vi "thermal_optical_capture_12.vi"() -> ()   [LabVIEW 2025]
panel:
  out "Optical saving error":errorcluster
  out "Thermal Preview":T1(plugin-control)
  in  "Stop Preview":bool
  out "Times between Frames":u32
  in  "STOP ACQUISITION":bool
  out "Optical Frame Out":string
  out "Optical Preview":T1(plugin-control)
  in  "Focus":dbl(slide) scale=0.0..100.0
  out "Thermal Frame Out":string
  in  "Output Folder":path
  in  "thermal capture interval (s)":dbl
  in  "Flag Button":bool
  in  "Stop & Save":bool
  in  "Record":bool
  # "Thermal Record"
  # "(Enter \"28\")"
  # "^ append to base data folder \"...\\test_n\\raw\" for nth recording"
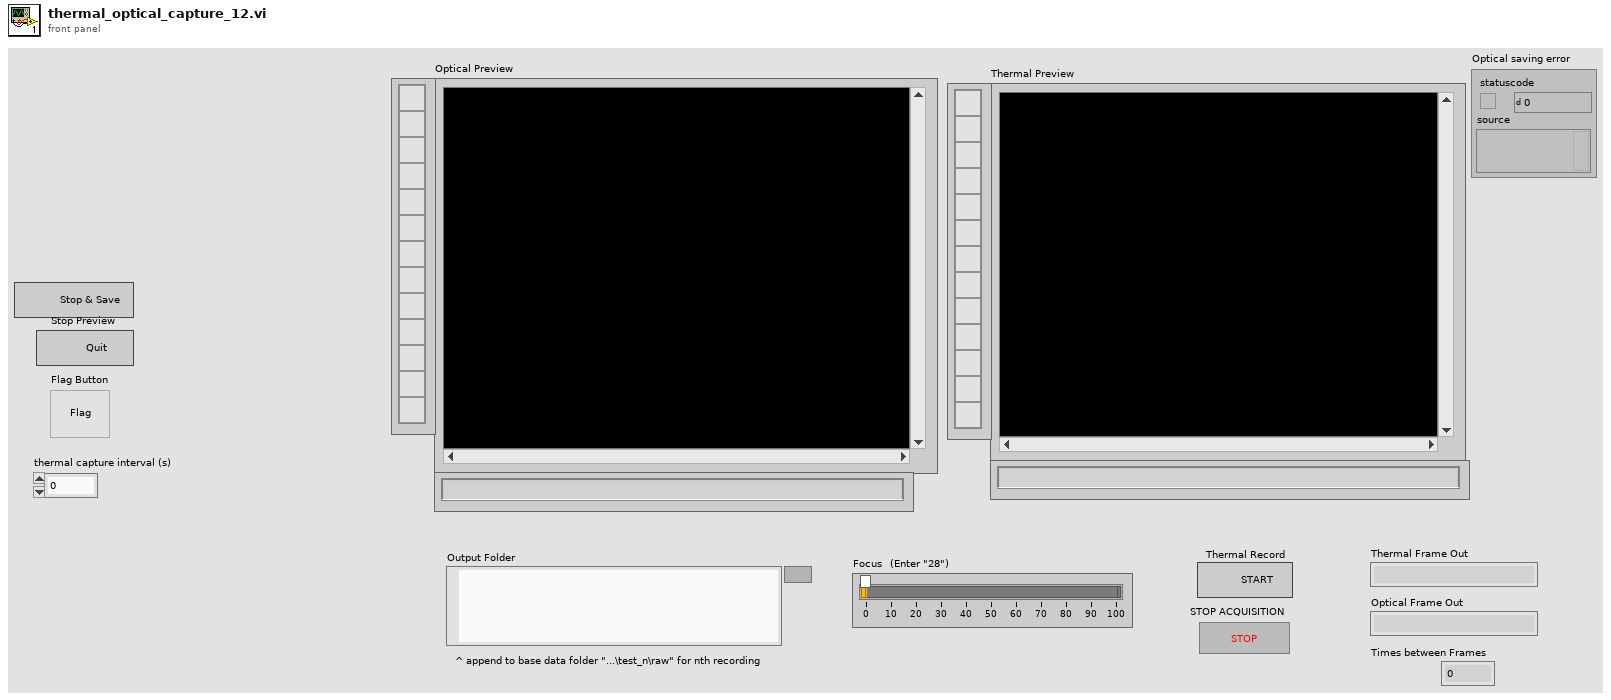
[diagram p1: front panel]
types:
  T1 = typedef "IMAQ Image.ctl" = refnum<image>
  T2 = enum16{"open", "replace", "create", "open or create", "replace or create", "replace or create with confirmation"}
  T3 = enum16{"big-endian, network order", "native, host order", "little-endian"}
  T4 = typedef "Image Type" = u32
  T5 = enum16{"Standard", "Buffered", "CRLF", "Immediate"}
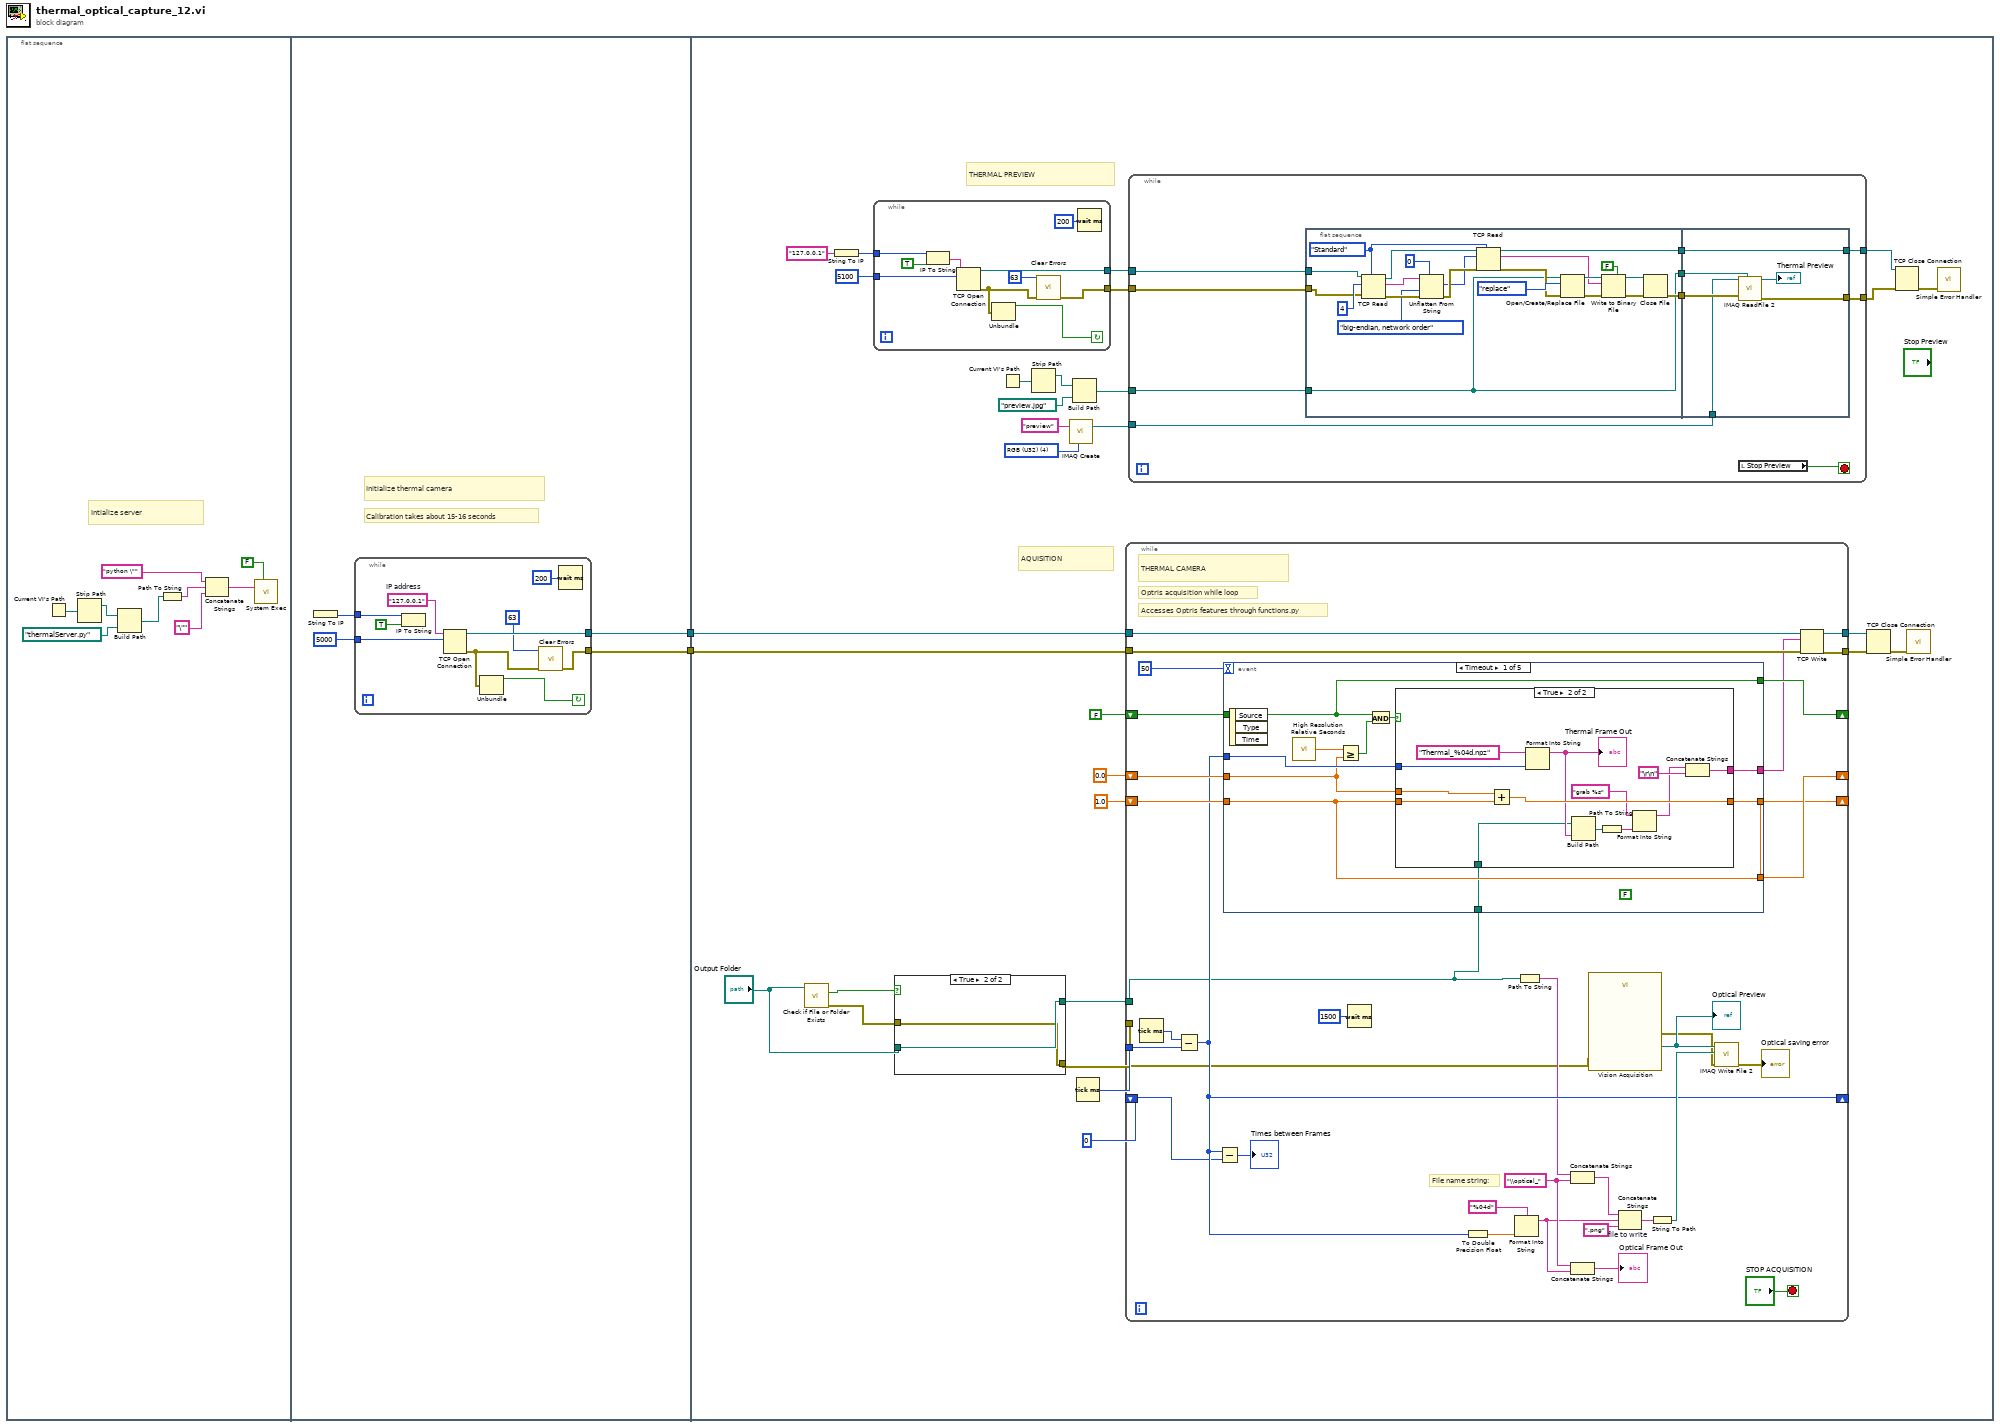
[diagram p0: block diagram]
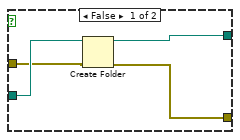
[diagram p2: hidden frame]
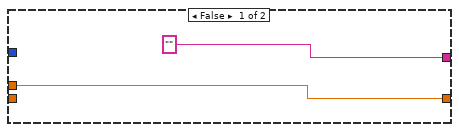
[diagram p3: hidden frame]
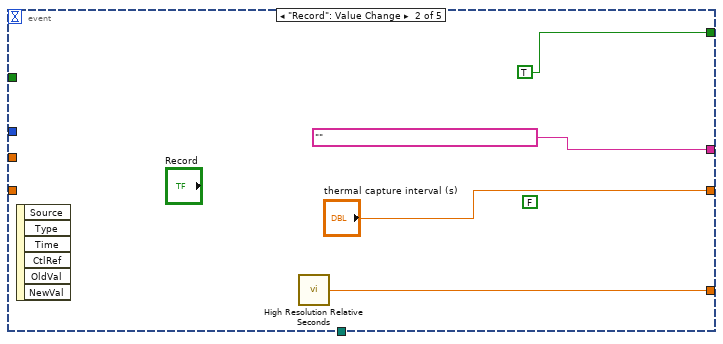
[diagram p4: hidden frame]
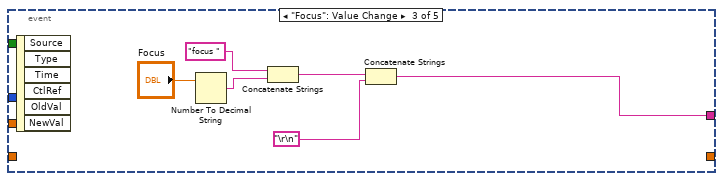
[diagram p5: hidden frame]
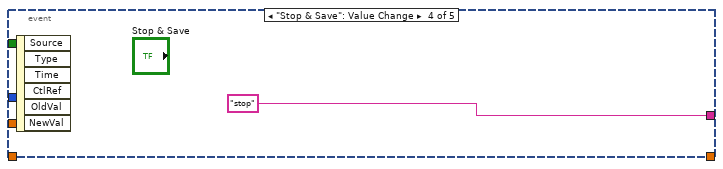
[diagram p6: hidden frame]
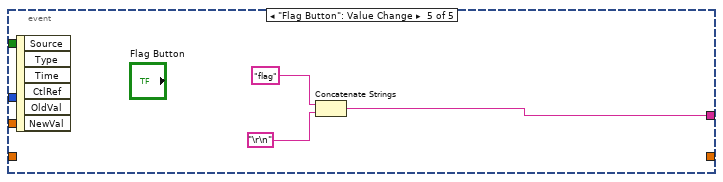
[diagram p7: hidden frame]
diagram:
  n1 = flat-sequence {
    tunnel: [w13] -> w2
    tunnel: [w12] -> w1
    tunnel: w1 -> [w52]
    tunnel: w2 -> [w51]
    frame #0 {
      # "Intialize server"
      n2 = Current VI's Path() -> (path=w6:path)
      n3 = Strip Path(path=w6) -> (stripped path=w7:path)  [unwired: 1 out]
      n4 = Build Path(base path=w7, name or relative path=path "thermalServer.py") -> (appended path=w4:path)
      n5 = Path To String(path=w4) -> (string=w10:string)
      n6 = Concatenate Strings("python \"" ("string"), w10, "\"" ("string")) -> (w9:string)
      n7 = call <vilib>:"System Exec.vi"("wait until completion? (T)"=FALSE, "command line"=w9) -> ()  [unwired: 6 in, 4 out]
    }
    frame #1 {
      # "Initialize thermal camera"
      # "Calibration takes about 15-16 seconds"
      n8 = String To IP() -> (0:w15:u32)  [unwired: 1 in]
      n9 = while {
        tunnel: [w20] -> w13
        tunnel: [w25] -> w12
        tunnel: w15 -> [w24]
        tunnel: u16 5000 ("remote port or service name") -> [w22]
        stop <- w17 continue-if-true
        w16 = "127.0.0.1"  # IP address
        n10 = IP To String(1:TRUE ("dot notation? (F)"), 2:w24) -> ()  [unwired: 1 out]
        n11 = TCP Open Connection(address=w16, remote port or service name=w22) -> (connection ID=w25:refnum<k5>, error out=w21:errorcluster)  [unwired: 3 in]
        n12 = Unbundle(w21) -> ("status"=w17:bool)  [unwired: 2 out]
        n13 = call <vilib>:"Clear Errors.vi"("error in (no error)"=w21, "specific error code to clear (0: all)"=63) -> ("error out"=w20:errorcluster)  [unwired: 4 in, 1 out]
        n14 = Wait (ms)(milliseconds to wait=u32 200) -> ()  [unwired: 1 out]
      }
    }
    frame #2 {
      w36 = T4 4 items=["Grayscale (U8)", "Grayscale (I16)", "Grayscale (SGL)", "Complex (CSG)", "RGB (U32)", "HSL (U32)", "RGB (U64)", "Grayscale (U16)"] ("Image Type")
      # "THERMAL PREVIEW"
      # "AQUISITION"
      n15 = call <vilib>:"Check if File or Folder Exists.vi"("path"="Output Folder") -> ("error out"=w27:errorcluster, "file or folder exists?"=w30:bool)  [unwired: 8 in, 1 out]
      n16 = String To IP(1:"127.0.0.1" ("name")) -> (0:w35:u32)
      n17 = while {
        tunnel: w35 -> [w71]
        tunnel: [w65] -> w34
        tunnel: [w69] -> w33
        tunnel: u16 5100 ("remote port or service name") -> [w67]
        stop <- w62 continue-if-true
        n18 = IP To String(1:TRUE ("dot notation? (F)"), 2:w71) -> (0:w70:string)
        n19 = TCP Open Connection(address=w70, remote port or service name=w67) -> (connection ID=w69:refnum<k5>, error out=w66:errorcluster)  [unwired: 3 in]
        n20 = Unbundle(w66) -> ("status"=w62:bool)  [unwired: 2 out]
        n21 = call <vilib>:"Clear Errors.vi"("error in (no error)"=w66, "specific error code to clear (0: all)"=63) -> ("error out"=w65:errorcluster)  [unwired: 4 in, 1 out]
        n22 = Wait (ms)(milliseconds to wait=u32 200) -> ()  [unwired: 1 out]
      }
      n23 = case shown="True" w30 {
        tunnel: "Output Folder" -> [w59 w61]
        tunnel: [w58 w61] -> w28
        tunnel: w27 -> [w57 w60]
        tunnel: [w56 w60] -> w26
        frame False {
          n24 = Create Folder(path (use dialog)=w59, error in=w57) -> (created path=w58:path, error out=w56:errorcluster)  [unwired: 1 in, 1 out]
        }
        frame True {
        }
      }
      n25 = Current VI's Path() -> (path=w44:path)
      n26 = Strip Path(path=w44) -> (stripped path=w45:path)  [unwired: 1 out]
      n27 = call "IMAQ Create"("Image Name"="preview", "Image Type"=w36) -> ("New Image"=w40:T1)  [unwired: 3 in, 1 out]
      n28 = Build Path(base path=w45, name or relative path=path "preview.jpg") -> (appended path=w43:path)
      n29 = Tick Count (ms)() -> (millisecond timer value=w47:u32)
      n30 = while {
        tunnel: [w143] -> w53
        tunnel: [w142] -> w54
        tunnel: w52 -> [w141]
        tunnel: w51 -> [w140]
        shift-right: [w139] -> _
        shift-left: 0.0 -> [w135]
        shift-right: [w136] -> _
        shift-left: 1.0 -> [w133]
        shift-right: [w137] -> _
        shift-left: FALSE -> [w134]
        tunnel: w47 -> [w118]
        shift-right: [w117] -> _
        shift-left: u32 0 -> [w116]
        tunnel: w28 -> [w112]
        tunnel: w26 -> [w113]
        stop <- "STOP ACQUISITION" stop-if-true
        w127 = "\\optical_" ("string")
        # "File name string:"
        # "THERMAL CAMERA"
        # "Optris acquisition while loop"
        # "Accesses Optris features through functions.py"
        n31 = Tick Count (ms)() -> (millisecond timer value=w119:u32)
        n32 = Subtract(x=w119, y=w118) -> (x-y=w117:u32)
        n33 = Subtract(x=w117, y=w116) -> (x-y=→"Times between Frames":u32)
        n34 = event shown="[0] Timeout" {
          selector: _ -> [_ _ _ _ _]
          dyn-events: _ -> [_ _ _ _ _]
          timeout: 50 -> [_ _ _ _ _]
          tunnel: [w149 "" w173 "stop" w182] -> w132
          tunnel: w117 -> [w150 _ _ _ _]
          tunnel: [w147 w172 _ _ _] -> w139
          tunnel: [w145 TRUE _ _ _] -> w137
          tunnel: [w146 "thermal capture interval (s)" _ _ _] -> w136
          tunnel: w135 -> [w148 _ _ _ _]
          tunnel: w134 -> [w145 _ _ _ _]
          tunnel: w133 -> [w146 _ _ _ _]
          tunnel: w112 -> [w144 _ _ _ _]
          event Timeout {
            (unwired) FALSE
            n35 = event-data() -> ()  [unwired: 1 in, 3 out]
            n36 = call <vilib>:"High Resolution Relative Seconds.vi"() -> ("relative seconds"=w153:dbl)
            n37 = Greater Or Equal?(x=w153, y=w148) -> (x >= y?=w152:bool)
            n38 = And(x=w145, y=w152) -> (x .and. y?=w151:bool)
            n39 = case shown="True" w151 {
              tunnel: w150 -> [_ w166]
              tunnel: ["" w167] -> w149
              tunnel: w148 -> [w154 w165]
              tunnel: w146 -> [_ w164]
              tunnel: [w154 w163] -> w147
              tunnel: w144 -> [_ w156]
              frame False {
              }
              frame True {
                n40 = Add(x=w165, y=w164) -> (x+y=w163:dbl)
                n41 = Format Into String(format string="Thermal_%04d.npz", w166) -> (resulting string=w157:string)  [unwired: 2 in, 1 out]
                "Thermal Frame Out" <- w157
                n42 = Build Path(base path=w156, name or relative path=w157) -> (appended path=w161:path)
                n43 = Path To String(path=w161) -> (string=w159:string)
                n44 = Format Into String(format string="grab %s", w159) -> (resulting string=w158:string)  [unwired: 2 in, 1 out]
                n45 = Concatenate Strings(w158, "\r\n") -> (w167:string)
              }
            }
          }
          event "Record": Value Change {
            (unwired) FALSE
            n46 = event-data() -> ()  [unwired: 1 in, 6 out]
            n47 = call <vilib>:"High Resolution Relative Seconds.vi"() -> ("relative seconds"=w172:dbl)
          }
          event "Focus": Value Change {
            n48 = event-data() -> ()  [unwired: 1 in, 6 out]
            n49 = Number To Decimal String(number="Focus") -> (decimal integer string=w178:string)  [unwired: 1 in]
            n50 = Concatenate Strings("focus ", w178) -> (w175:string)
            n51 = Concatenate Strings(w175, "\r\n") -> (w173:string)
          }
          event "Stop & Save": Value Change {
            n52 = event-data() -> ()  [unwired: 1 in, 6 out]
          }
          event "Flag Button": Value Change {
            n53 = event-data() -> ()  [unwired: 1 in, 6 out]
            n54 = Concatenate Strings("flag", "\r\n") -> (w182:string)
          }
        }
        n55 = Wait (ms)(milliseconds to wait=u32 1500) -> ()  [unwired: 1 out]
        n56 = To Double Precision Float(number=w117) -> (double precision float=w125:dbl)
        n57 = Format Into String(format string="%04d" ("time format string (%c)"), w125) -> (resulting string=w123:string)  [unwired: 2 in, 1 out]
        n58 = Path To String(path=w112) -> (string=w114:string)
        n59 = Concatenate Strings(w114, w127) -> (w128:string)
        n60 = Concatenate Strings(w127, w123) -> (→"Optical Frame Out":string)
        n61 = call "Vision Acquisition"("error in"=w113) -> ("Image Out"=w131:T1, "error out"=w111:errorcluster)  [unwired: 25 in]
        "Optical Preview" <- w131
        n62 = Concatenate Strings "file to write"(w128, w123, ".png" ("string")) -> (w130:string)
        n63 = String To Path(string=w130) -> (path=w124:path)
        n64 = call-poly "IMAQ Write File 2"("error in (no error)"=w111, "File Path"=w124, "Image"=w131) -> ("error out"=→"Optical saving error":errorcluster)  [unwired: 7 in, 1 out]
        n65 = TCP Write(connection ID=w141, data in=w132, error in (no error)=w140) -> (connection ID out=w142:refnum<k5>, error out=w143:errorcluster)  [unwired: 1 in, 1 out]
      }
      n66 = while {
        tunnel: w40 -> [w76]
        tunnel: [w77] -> w41
        tunnel: [w81] -> w42
        tunnel: w43 -> [w79]
        tunnel: w34 -> [w74]
        tunnel: w33 -> [w73]
        stop <- w72 stop-if-true
        n67 = flat-sequence {
          tunnel: w79 -> [w85]
          tunnel: [w87] -> w80
          tunnel: [w86] -> w78
          tunnel: [w85] -> w75
          tunnel: w74 -> [w83]
          tunnel: w73 -> [w82]
          tunnel: [w109] -> w81
          tunnel: w80 -> [w109]
          tunnel: w78 -> [w108]
          tunnel: [w107] -> w77
          tunnel: w76 -> [w106]
          tunnel: w75 -> [w105]
          frame #0 {
            w96 = T5."Standard" ("mode (standard)")
            n68 = TCP Read(connection ID=w82, bytes to read=4, error in (no error)=w83, 7:w96) -> (connection ID out=w99:refnum<k5>, data out=w84:string, error out=w102:errorcluster)  [unwired: 1 in]
            n69 = Unflatten From String(type=0, binary string=w84, byte order (0:big-endian, network order)=T3."big-endian, network order", error in (no error)=w102) -> (value=w97:i32, error out=w98:errorcluster)  [unwired: 1 in, 1 out]
            n70 = TCP Read(connection ID=w99, bytes to read=w97, error in (no error)=w98, 7:w96) -> (connection ID out=w87:refnum<k5>, data out=w92:string, error out=w94:errorcluster)  [unwired: 1 in]
            n71 = Open/Create/Replace File(file path (use dialog)=w85, error in=w94, operation (0:open)=T2."replace") -> (refnum out=w93:refnum<file>, error out=w90:errorcluster)  [unwired: 3 in, 1 out]
            n72 = Write to Binary File(file (use dialog)=w93, data=w92, error in=w90, 5:FALSE ("prepend array or string size? (T)")) -> (refnum out=w88:refnum<file>, error out=w89:errorcluster)  [unwired: 2 in, 1 out]
            n73 = Close File(refnum=w88, error in=w89) -> (error out=w86:errorcluster)  [unwired: 1 out]
          }
          frame #1 {
            n74 = call "IMAQ ReadFile 2"("File Path"=w105, "error in (no error)"=w108, "Image"=w106) -> ("error out"=w107:errorcluster, "Image Out"=→"Thermal Preview":T1)  [unwired: 4 in, 3 out]
          }
        }
        n75 = local read "Stop Preview"() -> (w72:bool)
      }
      n76 = TCP Close Connection(connection ID=w54, error in (no error)=w53) -> (error out=w55:errorcluster)  [unwired: 1 in, 1 out]
      n77 = TCP Close Connection(connection ID=w42, error in (no error)=w41) -> (error out=w39:errorcluster)  [unwired: 1 in, 1 out]
      n78 = call <vilib>:"Simple Error Handler.vi"("error in (no error)"=w55) -> ()  [unwired: 4 in, 5 out]
      n79 = call <vilib>:"Simple Error Handler.vi"("error in (no error)"=w39) -> ()  [unwired: 4 in, 5 out]
    }
  }
